vi "VIH Constant - Examples Folder.vi"(11 "append path":path) -> (3 "Examples folder":path)   [LabVIEW 2014]
doc: "::: VI Helpeks :::\nCopyright (c) 2000-2026 Konstantin Shifershteyn. All rights reserved."
panel:
  # "VI Helpeks\nCopyright (c) 2012-2026 Konstantin Shifershteyn"
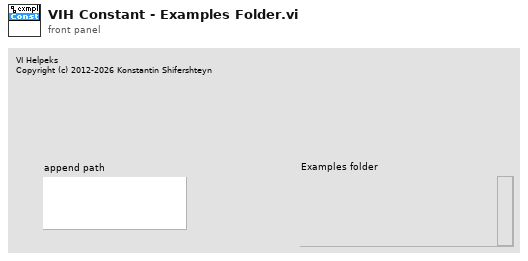
[diagram p1: front panel]
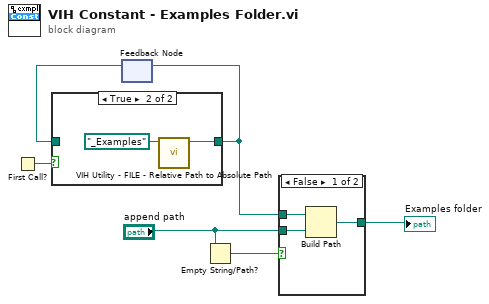
[diagram p0: block diagram]
diagram:
  n1 = First Call?() -> (First Call?: T/F=w3:bool)
  n2 = feedback #1() -> (w1:path)  [unwired: 1 in]
  n3 = case shown="True" w3 {
    tunnel: [w7 w8] -> w2
    tunnel: w1 -> [w7 _]
    frame False {
    }
    frame True {
      n4 = call "VIH Utility - FILE - Relative Path to Absolute Path.vi"("Path"=path "_Examples") -> ("Path out"=w8:path)  [unwired: 9 in, 1 out]
    }
  }
  n5 = feedback-in #1(w2) -> ()
  n6 = Empty String/Path?(string/path="append path") -> (empty?=w4:bool)
  n7 = case shown="False" w4 {
    tunnel: w2 -> [w12 w13]
    tunnel: "append path" -> [w11 _]
    tunnel: [w10 w13] -> w5
    frame False {
      n8 = Build Path(base path=w12, name or relative path=w11) -> (appended path=w10:path)
    }
    frame True {
    }
  }
  "Examples folder" <- w5
